vi "ImageAcquisition_16.vi"() -> ()   [LabVIEW 2025]
uses:
  <vilib>/vision/driver/IMAQdx.llb/IMAQdx Acquisition Mode.ctl
  <vilib>/vision/driver/NI_Vision_Acquisition_Software.lvlib
panel:
  out "Image":T1(plugin-control)
  out "error out":errorcluster
  out "Times between Frames":u32
  in  "Output Folder":path
  in  "Stop":bool
  in  "Camera Name":refnum<k21> caption="IMAQdx Session"
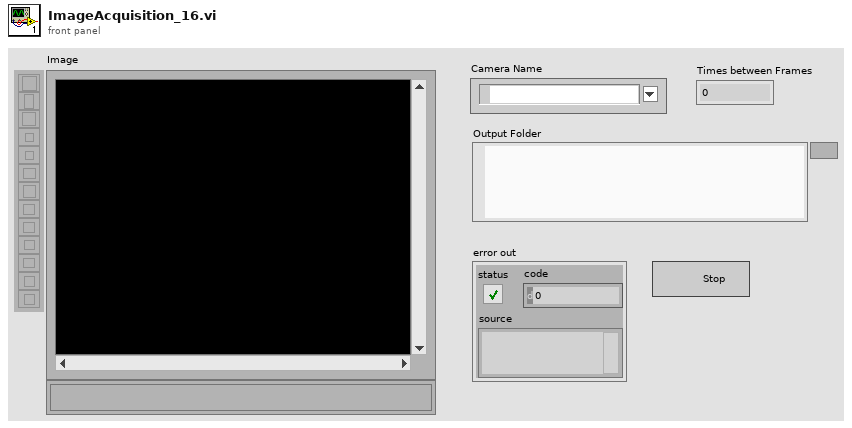
[diagram p1: front panel]
types:
  T1 = typedef "IMAQ Image.ctl" = refnum<image>
  T2 = typedef "Image Type" = u32
  T3 = typedef "NI_Vision_Acquisition_Software.lvlib/IMAQdx Acquisition Mode.ctl" = enum32{"One Shot", "Continuous"}
  T4 = typedef "IMAQdx.ctl" = refnum<k21>
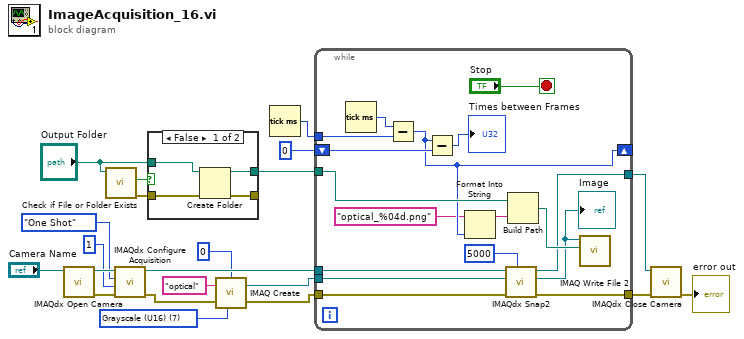
[diagram p0: block diagram]
diagram:
  w2 = T2 7 items=["Grayscale (U8)", "Grayscale (I16)", "Grayscale (SGL)", "Complex (CSG)", "RGB (U32)", "HSL (U32)", "RGB (U64)", "Grayscale (U16)"] ("Image Type")
  n1 = call <vilib>:"IMAQdx Open Camera.vi"("Session In"="Camera Name") -> ("error out"=w12:errorcluster, "Session Out"=w13:T4)  [unwired: 9 in]
  n2 = call <vilib>:"Check if File or Folder Exists.vi"("path"="Output Folder") -> ("error out"=w19:errorcluster, "file or folder exists?"=w21:bool)  [unwired: 8 in, 1 out]
  n3 = call <vilib>:"IMAQdx Configure Acquisition.vi"("error in"=w12, "Number of Buffers"=u32 1, "Continuous?"=IMAQdx_Acquisition_Mode."One Shot", "Session In"=w13) -> ("error out"=w5:errorcluster, "Session Out"=w7:T4)  [unwired: 6 in]
  n4 = case shown="False" w21 {
    tunnel: "Output Folder" -> [w25 w27]
    tunnel: [w24 w27] -> w18
    tunnel: w19 -> [w23 w26]
    tunnel: [w22 w26] -> _
    frame False {
      n5 = Create Folder(path (use dialog)=w25, error in=w23) -> (created path=w24:path, error out=w22:errorcluster)  [unwired: 1 in, 1 out]
    }
    frame True {
    }
  }
  n6 = call "IMAQ Create"("Border Size"=0, "Image Name"="optical", "Image Type"=w2, "error in (no error)"=w5) -> ("New Image"=w6:T1, "error out"=w4:errorcluster)  [unwired: 1 in]
  n7 = Tick Count (ms)() -> (millisecond timer value=w17:u32)
  n8 = while {
    tunnel: w18 -> [w44]
    tunnel: w17 -> [w42]
    shift-right: [w39] -> _
    shift-left: u32 0 -> [w40]
    tunnel: w7 -> [w31]
    tunnel: [w35] -> w15
    tunnel: [w34] -> w14
    tunnel: w4 -> [w33]
    tunnel: w6 -> [w30]
    stop <- "Stop" stop-if-true
    n9 = Tick Count (ms)() -> (millisecond timer value=w43:u32)
    n10 = Subtract(x=w43, y=w42) -> (x-y=w39:u32)
    n11 = Subtract(x=w39, y=w40) -> (x-y=→"Times between Frames":u32)
    n12 = Format Into String(format string="optical_%04d.png", w39) -> (resulting string=w38:string)  [unwired: 2 in, 1 out]
    n13 = call <vilib>:"IMAQdx Snap2.vi"("Timeout (ms)"=5000, "error in"=w33, "Image In"=w30, "Session In"=w31) -> ("error out"=w34:errorcluster, "Image Out"=w28:T1, "Session Out"=w35:T4)  [unwired: 5 in]
    "Image" <- w28
    n14 = Build Path(base path=w44, name or relative path=w38) -> (appended path=w36:path)
    n15 = call-poly "IMAQ Write File 2"("File Path"=w36, "Image"=w28) -> ()  [unwired: 8 in, 2 out]
  }
  n16 = call <vilib>:"IMAQdx Close Camera.vi"("error in"=w14, "Session In"=w15) -> ("error out"=→"error out":errorcluster)  [unwired: 9 in]
